vi "Create Message Accessors.vi"(5 "enum parameters":T1[](array[typedef]), 7 "message parameters":T2[](array[typedef]), 8 "error in (no error)":errorcluster, 11 "library in":refnum<vi>) -> (0 "error out":errorcluster, 3 "library out":refnum<vi>)   [LabVIEW 2019, in "gRPC Template Creation Utility.lvlib"]
uses:
  gRPC Template Creation Utility.lvlib
  TypeDefs/Message Metadata (Scripting).ctl
  TypeDefs/Message Element Metadata (Scripting).ctl
  TypeDefs/Message Element Type.ctl
  TypeDefs/Enum Metadata (Scripting).ctl
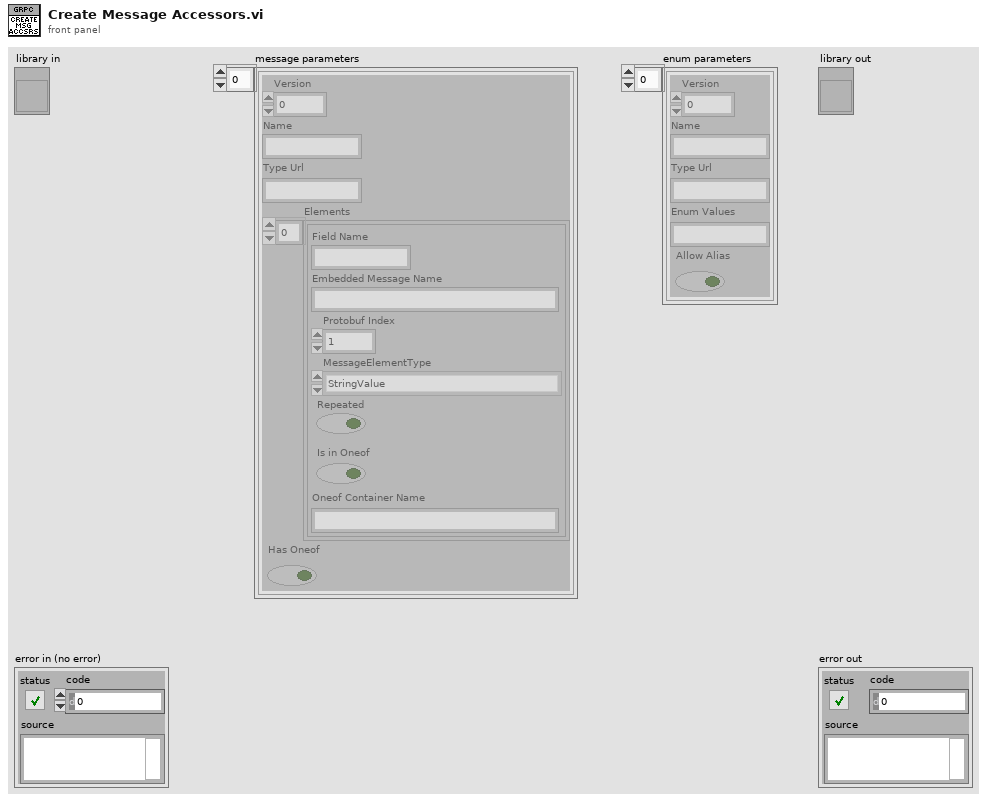
[diagram p1: front panel]
types:
  T1 = typedef "gRPC Template Creation Utility.lvlib/Enum Metadata (Scripting).ctl" = cluster{"Version":i32, "Name":string, "Type Url":string, "Enum Values":string, "Allow Alias":bool}
  T2 = typedef "gRPC Template Creation Utility.lvlib/Message Metadata (Scripting).ctl" = cluster{"Version":i32, "Name":string, "Type Url":string, "Elements":T3[], "Has Oneof":bool}
  T3 = typedef "gRPC Template Creation Utility.lvlib/Message Element Metadata (Scripting).ctl" = cluster{"Field Name":string, "Embedded Message Name":string, "Protobuf Index":i32, "MessageElementType":T4, "Repeated":bool, "Is in Oneof":bool, "Oneof Container Name":string}
  T4 = typedef "gRPC Template Creation Utility.lvlib/Message Element Type.ctl" = enum32{"Int32Value", "FloatValue", "DoubleValue", "BoolValue", "StringValue", "MessageValue", "Int64Value", "UInt32Value", "UInt64Value", "EnumValue", "Bytes", "Fixed64", "Fixed32", "SFixed64", "SFixed32", "SInt64", "SInt32"}
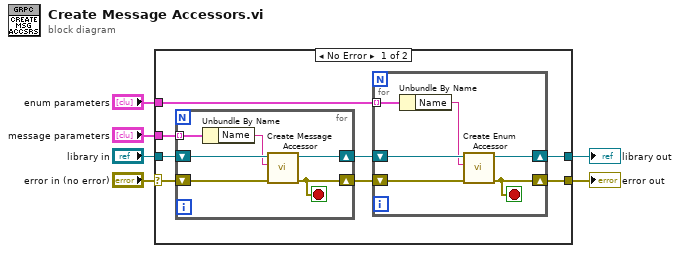
[diagram p0: block diagram]
diagram:
  n1 = case shown="No Error" "error in (no error)" {
    selector: "error in (no error)" -> [w13 w27]
    tunnel: [w7 w28] -> w6
    tunnel: "library in" -> [w12 w28]
    tunnel: [w10 w27] -> w4
    tunnel: "message parameters" -> [w14 _]
    tunnel: "enum parameters" -> [w9 _]
    frame No Error {
      n2 = for {
        shift-right: [w23] -> w11
        shift-left: w13 -> [w26]
        shift-right: [w24] -> w8
        shift-left: w12 -> [w25]
        tunnel: w14 -> [w22] mode=indexing
        stop <- w23 stop-if-true
        n3 = Unbundle By Name(w22) -> ("Name"=w21:string)
        n4 = call "Create Message Accessor.vi"("error in (no error)"=w26, "message name"=w21, "library in"=w25) -> ("error out"=w23:errorcluster, "library out"=w24:refnum<vi>)  [unwired: 7 in]
      }
      n5 = for {
        shift-right: [w16] -> w10
        shift-left: w11 -> [w17]
        shift-right: [w15] -> w7
        shift-left: w8 -> [w19]
        tunnel: w9 -> [w20] mode=indexing
        stop <- w16 stop-if-true
        n6 = Unbundle By Name(w20) -> ("Name"=w18:string)
        n7 = call "Create Enum Accessor.vi"("error in (no error)"=w17, "message name"=w18, "library in"=w19) -> ("error out"=w16:errorcluster, "library out"=w15:refnum<vi>)  [unwired: 7 in]
      }
    }
    frame Error {
    }
  }
  "library out" <- w6
  "error out" <- w4
